vi "[ce] Get All Refnums.vi"(8 "error in":errorcluster) -> (0 "error out":errorcluster, 1 "Size":i32, 2 "RefData":u64[](array[numeric]) format="%.0x", 3 "RefNums":u32[](array[numeric]) format="%.0x", 4 "error":i32)   [LabVIEW 2021]
doc: "::: CalcExpress Toolkit :::\nCopyright (c) 2000-2026 Konstantin Shifershteyn. All rights reserved."
uses:
  <vilib>/Utility/error.llb/DialogType.ctl
  cersrc/celveng32.dll
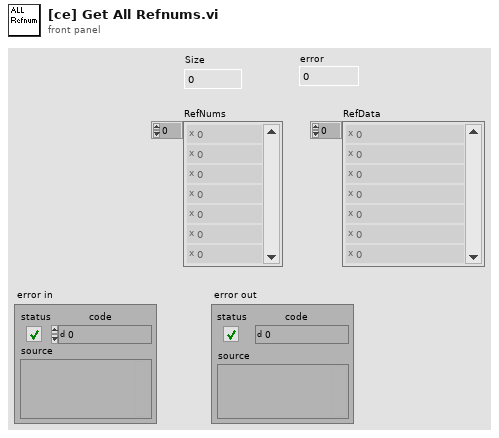
[diagram p1: front panel]
types:
  T1 = typedef "DialogType.ctl" = u16
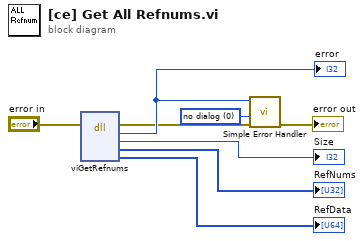
[diagram p0: block diagram]
diagram:
  w1 = T1 0 items=["no dialog", "OK message", "continue or stop message", "OK message + warnings", "continue/stop + warnings"] ("type of dialog (OK msg:1)")
  n1 = dll-call lib="C:/LV Projects/CalcExpress 40 LV2021/vi.lib/addons/CalcExpress/cersrc/celveng*.dll" fn="viGetRefnums"(error in="error in") -> (error out=w2:errorcluster, "return type"=w4:i32, "Size"=→"Size":i32, "RefNums"=→"RefNums":u32[], "RefData"=→"RefData":u64[])  [unwired: 5 in, 1 out]
  "error" <- w4
  n2 = call <vilib>:"Simple Error Handler.vi"("error code (no error:0)"=w4, "type of dialog (OK msg:1)"=w1, "error in (no error)"=w2) -> ("error out"=→"error out":errorcluster)  [unwired: 2 in, 4 out]
